vi "Test ISO8601 Decimal Strings.vi"(8 "error in (no error)":errorcluster) -> (0 "error out":errorcluster)   [LabVIEW 2013]
uses:
  <vilib>/addons/_JKI Toolkits/Caraya/classes/Assert/Assert True.vi
  <vilib>/addons/_JKI Toolkits/Caraya/classes/Assert/Assert.lvclass
  <vilib>/addons/_JKI Toolkits/Caraya/classes/Test/Test.lvclass
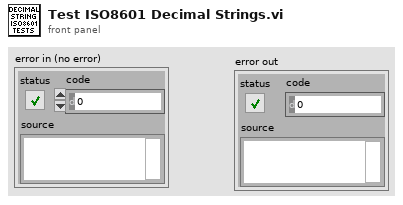
[diagram p1: front panel]
types:
  T1 = typedef "LVDateTimeRec.ctl" = cluster{"fractional second":dbl, "second":i32, "minute":i32, "hour":i32, "day of month":i32, "month":i32, "year":i32, "day of week":i32, "day of year":i32, "DST":i32}
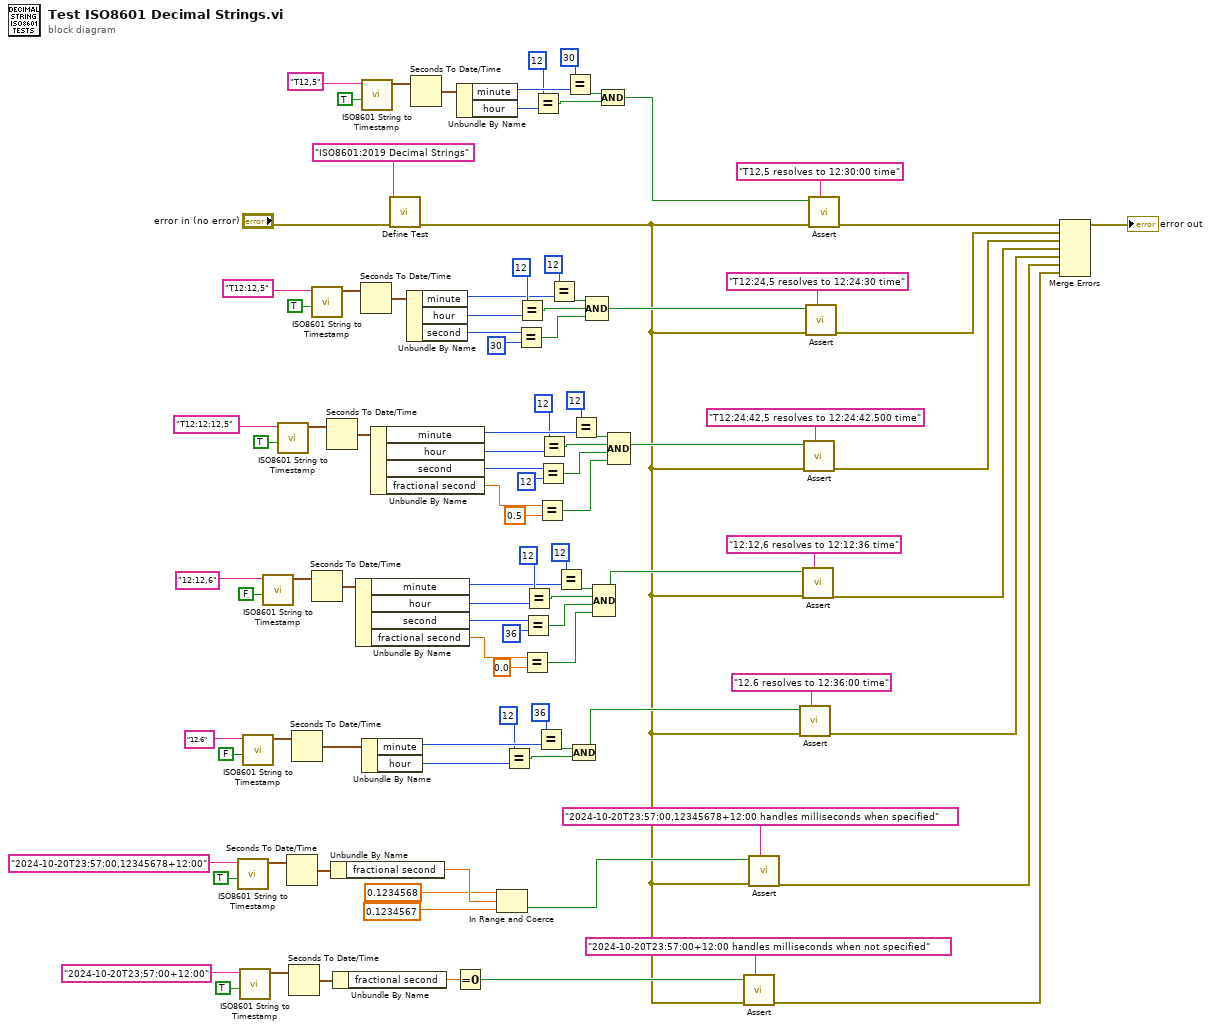
[diagram p0: block diagram]
diagram:
  n1 = call "ISO8601 String to Timestamp.vi"("Strict ISO? (T)"=TRUE, "ISO8601 String"="2024-10-20T23:57:00,12345678+12:00" ("Label (VI Title)")) -> ("Timestamp"=w17:timestamp)  [unwired: 7 in, 2 out]
  n2 = call "ISO8601 String to Timestamp.vi"("Strict ISO? (T)"=TRUE, "ISO8601 String"="2024-10-20T23:57:00+12:00" ("Label (VI Title)")) -> ("Timestamp"=w8:timestamp)  [unwired: 7 in, 2 out]
  n3 = call "ISO8601 String to Timestamp.vi"("Strict ISO? (T)"=FALSE, "ISO8601 String"="12.6" ("Label (VI Title)")) -> ("Timestamp"=w31:timestamp)  [unwired: 7 in, 2 out]
  n4 = call "ISO8601 String to Timestamp.vi"("Strict ISO? (T)"=FALSE, "ISO8601 String"="12:12,6" ("Label (VI Title)")) -> ("Timestamp"=w40:timestamp)  [unwired: 7 in, 2 out]
  n5 = call "ISO8601 String to Timestamp.vi"("Strict ISO? (T)"=TRUE, "ISO8601 String"="T12:12:12,5" ("Label (VI Title)")) -> ("Timestamp"=w67:timestamp)  [unwired: 7 in, 2 out]
  n6 = Seconds To Date/Time(time stamp (now)=w17) -> (date time rec=w18:T1)  [unwired: 1 in]
  n7 = Seconds To Date/Time(time stamp (now)=w8) -> (date time rec=w7:T1)  [unwired: 1 in]
  n8 = Seconds To Date/Time(time stamp (now)=w31) -> (date time rec=w30:T1)  [unwired: 1 in]
  n9 = call "ISO8601 String to Timestamp.vi"("Strict ISO? (T)"=TRUE, "ISO8601 String"="T12:12,5" ("Label (VI Title)")) -> ("Timestamp"=w81:timestamp)  [unwired: 7 in, 2 out]
  n10 = Seconds To Date/Time(time stamp (now)=w40) -> (date time rec=w41:T1)  [unwired: 1 in]
  n11 = Seconds To Date/Time(time stamp (now)=w67) -> (date time rec=w66:T1)  [unwired: 1 in]
  n12 = Unbundle By Name(w18) -> ("fractional second"=w15:dbl)
  n13 = Unbundle By Name(w7) -> ("fractional second"=w5:dbl)
  n14 = Unbundle By Name(w41) -> ("minute"=w42:i32, "hour"=w45:i32, "second"=w38:i32, "fractional second"=w49:dbl)
  n15 = Seconds To Date/Time(time stamp (now)=w81) -> (date time rec=w82:T1)  [unwired: 1 in]
  n16 = call "ISO8601 String to Timestamp.vi"("Strict ISO? (T)"=TRUE, "ISO8601 String"="T12,5" ("Label (VI Title)")) -> ("Timestamp"=w97:timestamp)  [unwired: 7 in, 2 out]
  n17 = Unbundle By Name(w30) -> ("minute"=w29:i32, "hour"=w26:i32)
  n18 = Unbundle By Name(w66) -> ("minute"=w65:i32, "hour"=w62:i32, "second"=w70:i32, "fractional second"=w54:dbl)
  n19 = call <vilib>:"Define Test.vi"("error in (no error)"="error in (no error)", "Label (VI Title)"="ISO8601:2019 Decimal Strings") -> ("error out"=w3:errorcluster)  [unwired: 8 in, 1 out]
  n20 = Unbundle By Name(w82) -> ("minute"=w83:i32, "hour"=w86:i32, "second"=w78:i32)
  n21 = Seconds To Date/Time(time stamp (now)=w97) -> (date time rec=w96:T1)  [unwired: 1 in]
  n22 = Equal To 0?(x=w5) -> (x = 0?=w4:bool)
  n23 = Unbundle By Name(w96) -> ("minute"=w95:i32, "hour"=w92:i32)
  n24 = In Range and Coerce(upper limit=0.1234568, x=w15, lower limit=0.1234567 ("upper limit")) -> (In Range?=w11:bool)  [unwired: 1 out]
  n25 = Equal?(x=12, y=w26) -> (x = y?=w25:bool)
  n26 = Equal?(x=w78, y=30 ("x")) -> (x = y?=w76:bool)
  n27 = Equal?(x=12, y=w86) -> (x = y?=w87:bool)
  n28 = Equal?(x=w49, y=0.0) -> (x = y?=w51:bool)
  n29 = Equal?(x=w38, y=36 ("x")) -> (x = y?=w37:bool)
  n30 = Equal?(x=12, y=w45) -> (x = y?=w46:bool)
  n31 = Equal?(x=12, y=w92) -> (x = y?=w91:bool)
  n32 = Equal?(x=36, y=w29) -> (x = y?=w24:bool)
  n33 = Equal?(x=w54, y=0.5) -> (x = y?=w52:bool)
  n34 = Equal?(x=w70, y=12 ("x")) -> (x = y?=w71:bool)
  n35 = Equal?(x=12, y=w62) -> (x = y?=w61:bool)
  n36 = Equal?(x=12, y=w83) -> (x = y?=w88:bool)
  n37 = Equal?(x=12, y=w42) -> (x = y?=w47:bool)
  n38 = Equal?(x=30, y=w95) -> (x = y?=w90:bool)
  n39 = Equal?(x=12, y=w65) -> (x = y?=w60:bool)
  n40 = Compound Arithmetic op=AND(w24, w25) -> (w21:bool)
  n41 = Compound Arithmetic op=AND(w88, w87, w76) -> (w74:bool)
  n42 = Compound Arithmetic op=AND(w47, w46, w37, w51) -> (w34:bool)
  n43 = Compound Arithmetic op=AND(w90, w91) -> (w89:bool)
  n44 = Compound Arithmetic op=AND(w60, w61, w71, w52) -> (w73:bool)
  n45 = call-poly <vilib>:"Assert.vi"("Label"="2024-10-20T23:57:00+12:00 handles milliseconds when not specified" ("x"), "error in (no error)"=w3, "True?"=w4) -> ("error out"=w2:errorcluster)  [unwired: 7 in, 1 out]
  n46 = call-poly <vilib>:"Assert.vi"("Label"="2024-10-20T23:57:00,12345678+12:00 handles milliseconds when specified" ("x"), "error in (no error)"=w3, "True?"=w11) -> ("error out"=w10:errorcluster)  [unwired: 7 in, 1 out]
  n47 = call-poly <vilib>:"Assert.vi"("Label"="12.6 resolves to 12:36:00 time" ("x"), "error in (no error)"=w3, "True?"=w21) -> ("error out"=w20:errorcluster)  [unwired: 7 in, 1 out]
  n48 = call-poly <vilib>:"Assert.vi"("Label"="12:12,6 resolves to 12:12:36 time" ("x"), "error in (no error)"=w3, "True?"=w34) -> ("error out"=w33:errorcluster)  [unwired: 7 in, 1 out]
  n49 = call-poly <vilib>:"Assert.vi"("Label"="T12:24:42,5 resolves to 12:24:42.500 time" ("x"), "error in (no error)"=w3, "True?"=w73) -> ("error out"=w57:errorcluster)  [unwired: 7 in, 1 out]
  n50 = call-poly <vilib>:"Assert.vi"("Label"="T12:24,5 resolves to 12:24:30 time" ("x"), "error in (no error)"=w3, "True?"=w74) -> ("error out"=w58:errorcluster)  [unwired: 7 in, 1 out]
  n51 = call-poly <vilib>:"Assert.vi"("Label"="T12,5 resolves to 12:30:00 time" ("x"), "error in (no error)"=w3, "True?"=w89) -> ("error out"=w59:errorcluster)  [unwired: 7 in, 1 out]
  n52 = Merge Errors(w59, w58, w57, w33, w20, w10, w2) -> (→"error out":errorcluster)
